vi "Simple Reader.vi"(8 "error in (no error)":errorcluster, 11 "SRS CTC100 Driver in":refnum<class "SRS CTC100 Driver.lvclass">) -> (0 "error out":errorcluster, 2 "Signals":dbl[](array[numeric]), 3 "SRS CTC100 Driver out":refnum<class "SRS CTC100 Driver.lvclass">)   [LabVIEW 2024, in "SRS CTC100 Driver.lvclass"]
uses:
  SRS CTC100 Driver.lvclass
  C:/Nano/fedor2026/NHMFL_Core/Libraries/Instruments/VISA Instrument/VISA Instrument.lvclass
  C:/Nano/fedor2026/NHMFL_Core/Libraries/Instruments/Temperature Controller Driver/Temperature Controller Driver.lvclass
  VISA Instrument/VISA Instrument.lvclass/VISA Instrument.ctl
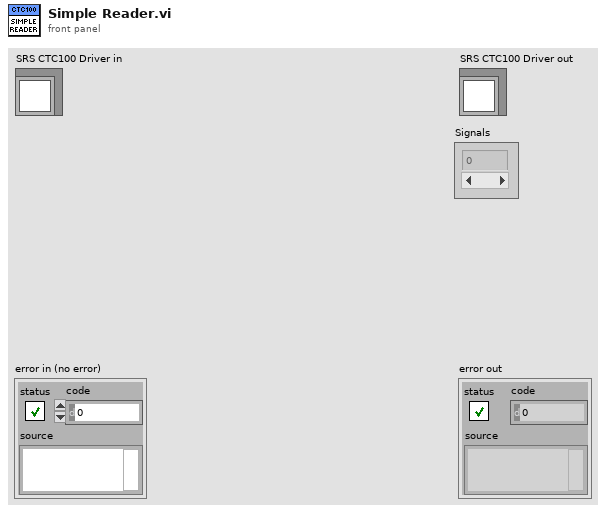
[diagram p1: front panel]
types:
  T1 = typedef "T controller configuration.ctl" = cluster{"Record Channels":string[], "Record raw signal":bool, "Set point":dbl, "Record heater":bool, "Ramp rate":dbl, "P":dbl, "I":dbl, "D":dbl, "Control":T2, "P manual":dbl, "Output #":i32}
  T2 = typedef "Control Mode.ctl" = enum16{"Off", "PID", "Ramp", "Manual", "Table"}
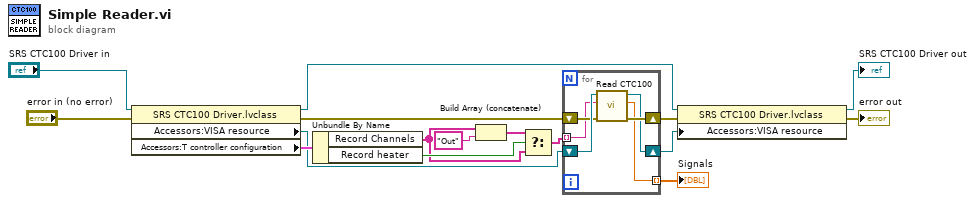
[diagram p0: block diagram]
diagram:
  n1 = property class="SRS CTC100 Driver.lvclass"(reference="SRS CTC100 Driver in", error in="error in (no error)") -> (reference out=w4:refnum<class "SRS CTC100 Driver.lvclass">, error out=w13:errorcluster, "Accessors:VISA resource"=w12:refnum<visa-resource-name>, "Accessors:T controller configuration"=w14:T1)
  n2 = Unbundle By Name(w14) -> ("Record Channels"=w7:string[], "Record heater"=w11:bool)
  n3 = Build Array (concatenate)(w7, "Out") -> (w9:string[])
  n4 = Select(t=w9, s=w11, f=w7) -> (s? t:f=w8:string[])
  n5 = for {
    shift-right: [w18] -> w5
    shift-left: w12 -> [w22]
    shift-right: [w19] -> w2
    shift-left: w13 -> [w21]
    tunnel: w8 -> [w20] mode=indexing
    tunnel: [w17] -> w6 mode=indexing
    n6 = call "Read CTC100.vi"("error in"=w21, "Read channel"=w20, "VISA resource name"=w22) -> ("error out"=w19:errorcluster, "Value out"=w17:dbl, "VISA resource name out"=w18:refnum<visa-resource-name>)  [unwired: 6 in]
  }
  "Signals" <- w6
  n7 = property class="SRS CTC100 Driver.lvclass"(reference=w4, error in=w2, "Accessors:VISA resource"=w5) -> (reference out=→"SRS CTC100 Driver out":refnum<class "SRS CTC100 Driver.lvclass">, error out=→"error out":errorcluster)
